vi "RemoteVI Check Next Free Port.vi"() -> (4 "labels":string[](array[string]), 6 "expected":string[](array[string]), 8 "actual":string[](array[string]), 10 "failures":i32)   [LabVIEW 2020]
doc: "Test support, generated by tests/caraya/build.py from tests/vectors/server-app.json (nextFreePort) - do not edit. Calls RemoteVI Next Free Port.vi once per vector: used and start as in the vector; the port is rendered as a decimal number. Outputs, one element per vector: labels (the vector's name), expected (rendered from the vector), actual (the VI's result rendered the same way), and failures, the number of vectors whose expected and actual differ."
uses:
  source/RemoteVI.lvlib
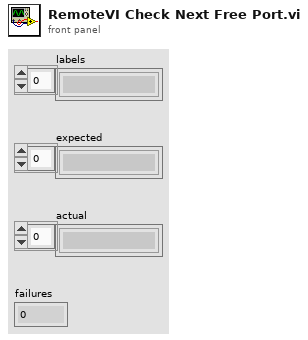
[diagram p1: front panel]
types:
  T1 = cluster{"name":string, "used":u16[], "start":u16, "expect":string}[]
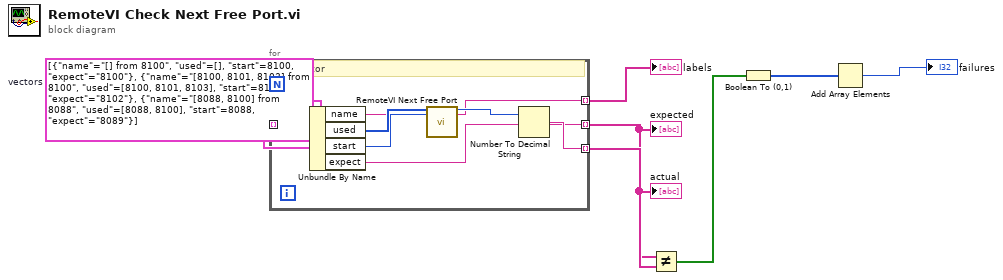
[diagram p0: block diagram]
diagram:
  w1 = T1 [{"name"="[] from 8100", "used"=[], "start"=8100, "expect"="8100"}, {"name"="[8100, 8101, 8103] from 8100", "used"=[8100, 8101, 8103], "start"=8100, "expect"="8102"}, {"name"="[8088, 8100] from 8088", "used"=[8088, 8100], "start"=8088, "expect"="8089"}]  # vectors
  n1 = for {
    tunnel: w1 -> [w8] mode=indexing
    tunnel: [w9] -> w2 mode=indexing
    tunnel: [w12] -> w3 mode=indexing
    tunnel: [w14] -> w4 mode=indexing
    # "One vector"
    n2 = Unbundle By Name(w8) -> ("name"=w9:string, "used"=w10:u16[], "start"=w11:u16, "expect"=w12:string)
    n3 = call "RemoteVI Next Free Port.vi"("used"=w10, "start"=w11) -> ("port"=w13:u16)  [unwired: 13 in]
    n4 = Number To Decimal String(number=w13) -> (decimal integer string=w14:string)  [unwired: 1 in]
  }
  "labels" <- w2
  "expected" <- w3
  "actual" <- w4
  n5 = Not Equal?(x=w3, y=w4) -> (x != y?=w5:bool[])
  n6 = Boolean To (0,1)(Boolean=w5) -> (0, 1=w6:i16[])
  n7 = Add Array Elements(numeric array=w6) -> (sum=→"failures":i16)
